vi "Load DAC Configuration.vi"(8 "error in":errorcluster, 10 "Config File refnum in":T1, 11 "DAC Traverse in":refnum<class "DAC Traverse.lvclass">) -> (0 "error out":errorcluster, 2 "Config File refnum out":T1, 3 "DAC Traverse out":refnum<class "DAC Traverse.lvclass">)   [LabVIEW 2019, in "DAC.lvlib" / "DAC Traverse.lvclass"]
uses:
  DAC Traverse.lvclass
  C:/Users/krio/Documents/LV_Projects/test-stand/App/DAC/DAC.lvclass
  <vilib>/Utility/config.llb/Config Data RefNum.ctl
  DAC.lvclass/DAC.ctl
  DAC Traverse.lvclass/DAC Traverse.ctl
  <vilib>/Utility/config.llb/Read Key (String).vi
  DAC.lvclass
  <vilib>/Utility/config.llb/NI_LVConfig.lvlib
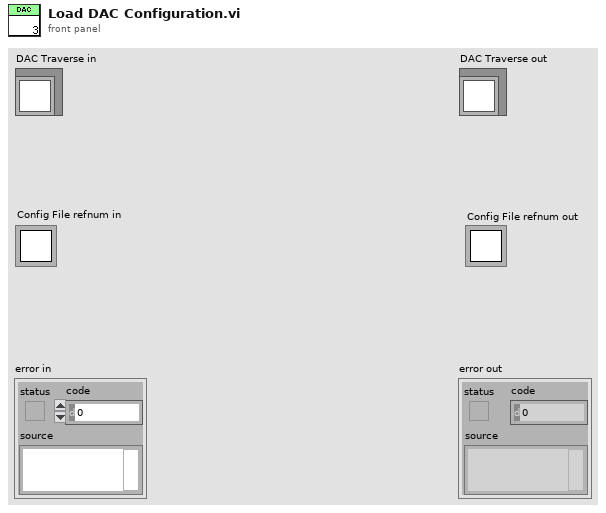
[diagram p1: front panel]
types:
  T1 = typedef "NI_LVConfig.lvlib/Config Data RefNum.ctl" = refnum<k1>
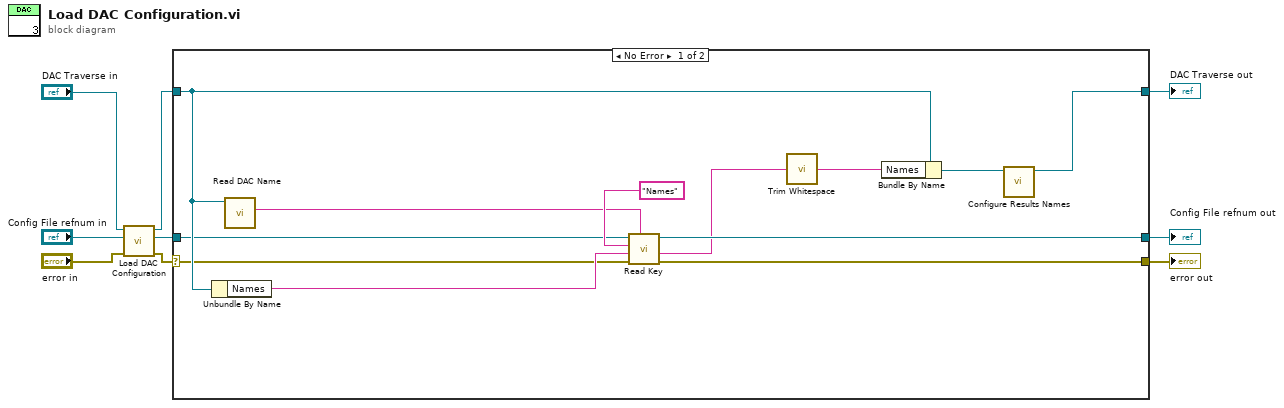
[diagram p0: block diagram]
diagram:
  n1 = call-parent "Load DAC Configuration.vi"("error in"="error in", "Config File refnum in"="Config File refnum in", "DAC in"="DAC Traverse in") -> ("error out"=w4:errorcluster, "Config File refnum out"=w5:T1, "DAC out"=w6:refnum<class "DAC Traverse.lvclass">)  [unwired: 6 in]
  n2 = case shown="No Error" w4 {
    selector: w4 -> [w14 w22]
    tunnel: [w12 w24] -> w3
    tunnel: w6 -> [w20 w24]
    tunnel: w5 -> [w15 w23]
    tunnel: [w17 w23] -> w2
    tunnel: [w18 w22] -> w1
    frame No Error {
      n3 = Unbundle By Name(w20) -> ("Names"=w19:string)
      n4 = call "Read DAC Name.vi"("DAC in"=w20) -> ("DAC Name"=w16:string)  [unwired: 8 in, 2 out]
      n5 = call-poly <vilib>:"Read Key.vi"("section"=w16, "error in (no error)"=w14, "default value"=w19, "key"="Names", "refnum"=w15) -> ("error out"=w18:errorcluster, "value"=w10:string, "refnum out"=w17:T1)  [unwired: 3 in, 1 out]
      n6 = call <vilib>:"Trim Whitespace.vi"("string"=w10) -> ("trimmed string"=w11:string)  [unwired: 1 in]
      n7 = Bundle By Name(cluster=w20, "Names"=w11) -> (w13:refnum<class "DAC Traverse.lvclass">)
      n8 = call "Configure Results Names.vi"("DAC Traverse in"=w13) -> ("DAC Traverse out"=w12:refnum<class "DAC Traverse.lvclass">)  [unwired: 9 in, 1 out]
    }
    frame Error {
    }
  }
  "error out" <- w1
  "DAC Traverse out" <- w3
  "Config File refnum out" <- w2
